vi "Wrapper.vi"(0 "measurement configuration":T1={"Vin SMU Channel"="0", "Range"=1.2, "Resolution in Digits"=4.5, "Voltage Config Str"="{\"Voltage Level\":2,\"Voltage Level Range\":6}", "Current Config Str"="{\"Current Limit\":0.01,\"Current Limit Range\":0.01}", "Vin SMU Pin"="Vcc", "Device Name Pin"="Vdd"} {"Resolution in Digits" items=["3 1/2"=3.5, "4 1/2"=4.5, "5 1/2"=5.5, "6 1/2"=6.5, "7 1/2"=7.5]}, 5 "Vin SMU":refnum<k15>="Dev1", 7 "Device Name":refnum<k15>="Dev1", 11 "error in":errorcluster) -> (4 "measurement results":T3={"Measurement "=0.0, "Signal Out of Range"=FALSE, "Measurement from SMU Str"="Empty", "Waveform Graph"=[0.0]} {"Measurement" format="%.6p"}, 15 "error out":errorcluster)   [LabVIEW 2021, in "Voltage Measurement.lvlib"]
uses:
  Voltage Measurement.lvlib
  Measurement Results.ctl
  Measurement Configuration.ctl
  <instrlib>/niDMM/nidmm.llb/niDMM Resolution in Digits.ctl
  MeasurementCore/Main_Voltage Measurement.lvlib
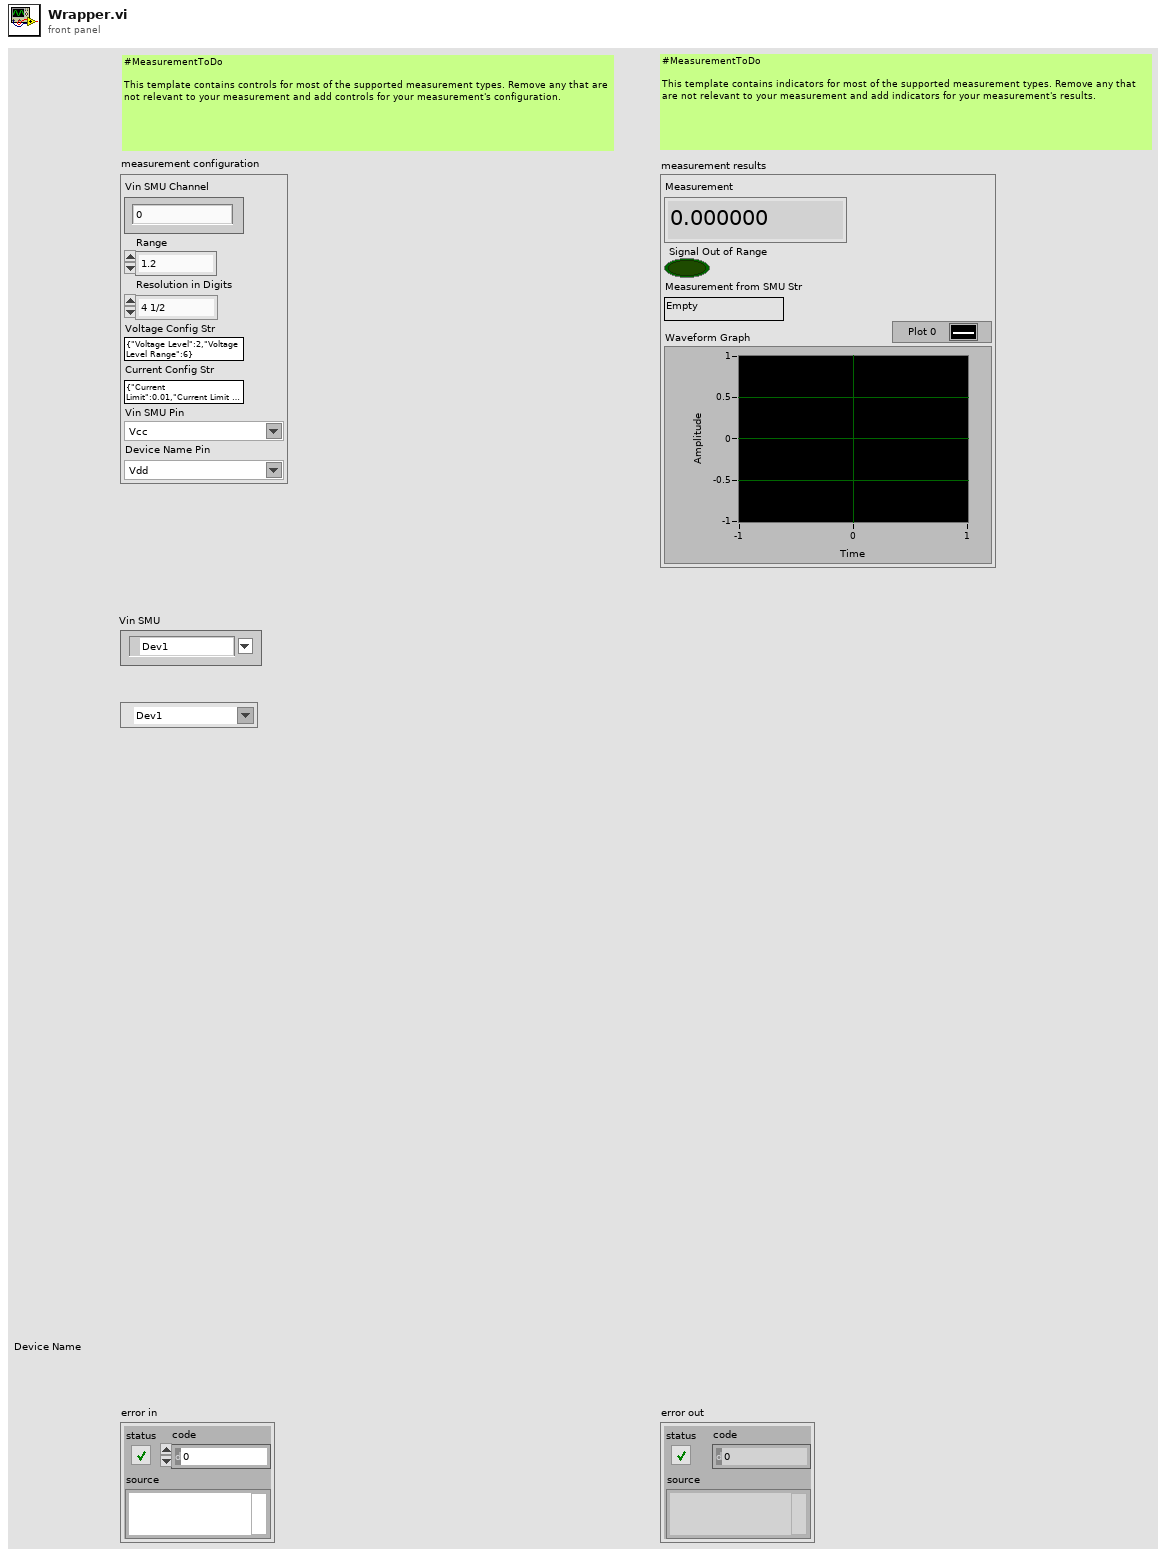
[diagram p1: front panel]
types:
  T1 = typedef "Voltage Measurement.lvlib/Measurement Configuration.ctl" = cluster{"Vin SMU Channel":string, "Range":dbl, "Resolution in Digits":T2, "Voltage Config Str":string, "Current Config Str":string, "Vin SMU Pin":string, "Device Name Pin":string}
  T2 = typedef "niDMM Resolution in Digits.ctl" = dbl
  T3 = typedef "Voltage Measurement.lvlib/Measurement Results.ctl" = cluster{"Measurement ":dbl, "Signal Out of Range":bool, "Measurement from SMU Str":string, "Waveform Graph":dbl[]}
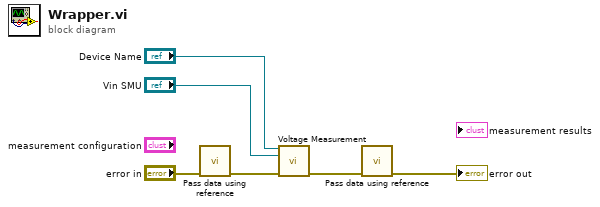
[diagram p0: block diagram]
diagram:
  n1 = call "Pass data using reference.vi"("error in"="error in") -> ("error out"=w3:errorcluster)  [unwired: 14 in]
  n2 = call "Voltage Measurement.vi"("Device Name"="Device Name", "Vin SMU"="Vin SMU", "error in"=w3) -> ("error out"=w2:errorcluster)  [unwired: 12 in]
  n3 = call "Pass data using reference.vi"("error in"=w2) -> ("error out"=→"error out":errorcluster)  [unwired: 14 in]
